vi "AM.vi"() -> ()   [LabVIEW 2021]
panel:
  out "demodulated":dynamicdata(graph)
  out "modulated":dynamicdata(graph)
  out "carrier":dynamicdata(graph)
  out "message":dynamicdata(graph)
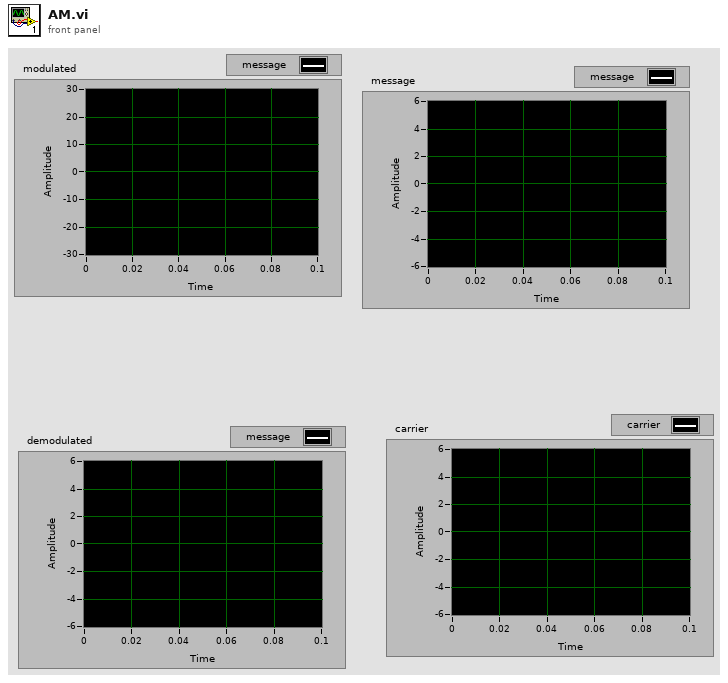
[diagram p1: front panel]
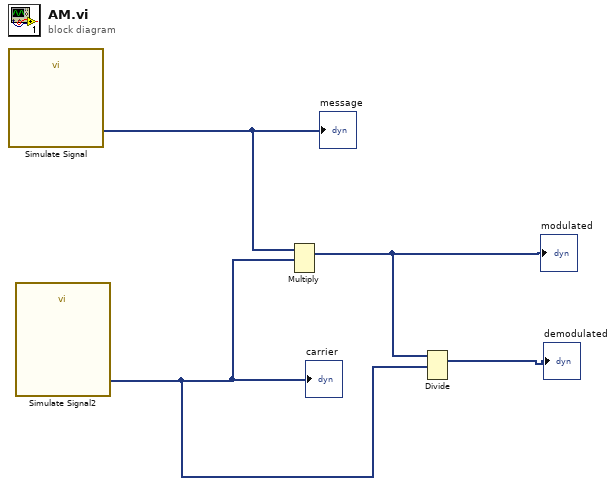
[diagram p0: block diagram]
diagram:
  n1 = call "Simulate Signal"() -> ("message"=w4:dynamicdata)  [unwired: 14 in, 1 out]
  "message" <- w4
  n2 = call "Simulate Signal2"() -> ("carrier"=w1:dynamicdata)  [unwired: 14 in, 1 out]
  "carrier" <- w1
  n3 = Multiply(1:w1, 2:w4) -> (0:w2:dynamicdata)  [unwired: 1 in, 1 out]
  "modulated" <- w2
  n4 = Divide(1:w1, 2:w2) -> (0:→"demodulated":dynamicdata)  [unwired: 1 in, 1 out]
